vi "Is String Constant a State Constant.vi"(8 "error in (no error)":errorcluster, 11 "GObj Refnum":refnum<vi>) -> (0 "error out":errorcluster, 2 "Is States Constant":bool, 3 "Add States to Queue":refnum<vi>)   [LabVIEW 2020, in "JKI State Machine API.lvlib"]
uses:
  JKI State Machine API.lvlib
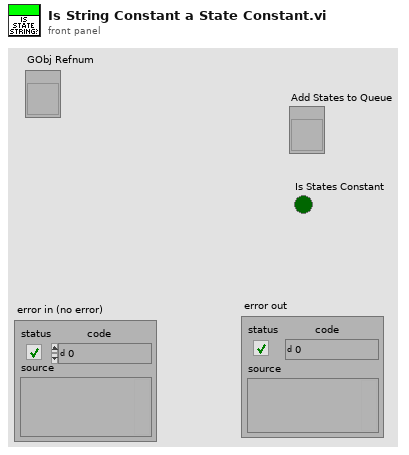
[diagram p1: front panel]
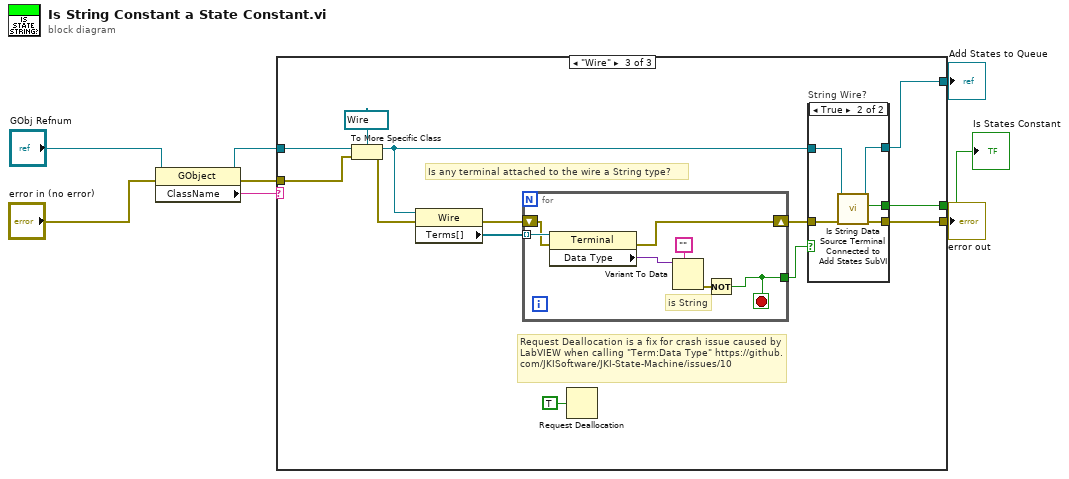
[diagram p0: block diagram]
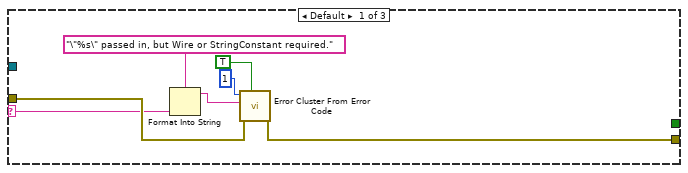
[diagram p2: hidden frame]
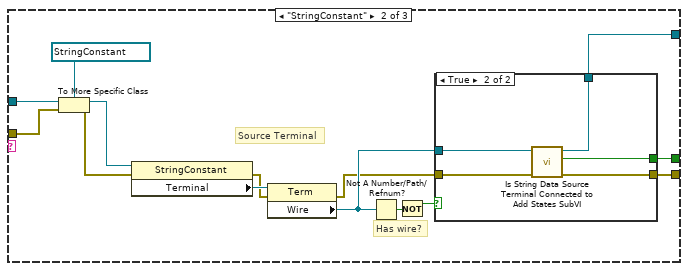
[diagram p3: hidden frame]
diagram:
  n1 = property class="GObject"(reference="GObj Refnum", error in="error in (no error)") -> (reference out=w4:refnum<vi>, error out=w2:errorcluster, "ClassName"=w1:string)
  n2 = case shown="\"Wire\"" w1 {
    selector: w1 -> [w13 _ _]
    tunnel: [w14 w29 w42] -> w8
    tunnel: [_ w28 w44] -> w7
    tunnel: [_ w27 w43] -> w6
    tunnel: w4 -> [_ w23 w46]
    tunnel: w2 -> [w15 w22 w45]
    frame Default {
      n3 = Format Into String(format string="\"%s\" passed in, but Wire or StringConstant required.", w13) -> (resulting string=w11:string)  [unwired: 2 in, 1 out]
      n4 = call <vilib>:"Error Cluster From Error Code.vi"("show call chain? (False)"=TRUE, "error in (no error)"=w15, "error message (\"\")"=w11, "error code (0)"=1) -> ("error out"=w14:errorcluster)  [unwired: 5 in]
    }
    frame "StringConstant" {
      # "Has wire?"
      # "Source Terminal"
      n5 = To More Specific Class(target class=refnum<vi> refnum ("StrCnst Refnum"), reference=w23, error in=w22) -> (specific class reference=w26:refnum<vi>, error out=w24:errorcluster)
      n6 = property class="StringConstant"(reference=w26, error in=w24) -> (error out=w17:errorcluster, "Terminal"=w21:refnum<vi>)  [unwired: 1 out]
      n7 = property class="Term"(reference=w21, error in=w17) -> (error out=w16:errorcluster, "Wire"=w18:refnum<vi>)  [unwired: 1 out]
      n8 = Not A Number/Path/Refnum?(number/path/refnum=w18) -> (NaN/Path/Refnum?=w20:bool)
      n9 = Not(x=w20) -> (.not. x?=w19:bool)
      n10 = case shown="True" w19 {
        tunnel: [w30 w35] -> w29
        tunnel: [_ w34] -> w28
        tunnel: w16 -> [w30 w33]
        tunnel: [_ w32] -> w27
        tunnel: w18 -> [_ w31]
        frame False {
        }
        frame True {
          n11 = call "Is String Data Source Terminal Connected to Add States SubVI.vi"("error in (no error)"=w33, "Wire"=w31) -> ("error out"=w35:errorcluster, "Connected to Add States?"=w34:bool, "Add States SubVI"=w32:refnum<vi>)  [unwired: 6 in, 1 out]
        }
      }
    }
    frame "Wire" {
      # "Request Deallocation is a fix for crash issue caused by LabVIEW when calling \"Term:Data Type\" https://github.com/JKISoftware/JKI-State-Machine/issues/10"
      # "Is any terminal attached to the wire a String type?"
      n12 = To More Specific Class(target class=refnum<vi> refnum ("Wire Refnum"), reference=w46, error in=w45) -> (specific class reference=w41:refnum<vi>, error out=w47:errorcluster)
      n13 = property class="Wire"(reference=w41, error in=w47) -> (error out=w40:errorcluster, "Terms[]"=w38:refnum<vi>[])  [unwired: 1 out]
      n14 = for {
        shift-right: [w59] -> w39
        shift-left: w40 -> [w60]
        tunnel: w38 -> [w61] mode=indexing
        tunnel: [w55] -> w37
        stop <- w55 stop-if-true
        # "is String"
        n15 = property class="Terminal"(reference=w61, error in=w60) -> (error out=w59:errorcluster, "Data Type"=w56:variant)  [unwired: 1 out]
        n16 = Variant To Data(type="" ("error in (no error)"), Variant=w56) -> (error out=w57:errorcluster)  [unwired: 1 in, 1 out]
        n17 = Not(x=w57) -> (.not. x?=w55:bool)
      }
      n18 = Request Deallocation(TRUE ("flag")) -> ()
      n19 = case "String Wire?" shown="True" w37 {
        tunnel: [_ w54] -> w44
        tunnel: [_ w53] -> w43
        tunnel: [w49 w52] -> w42
        tunnel: w41 -> [_ w51]
        tunnel: w39 -> [w49 w50]
        frame False {
        }
        frame True {
          n20 = call "Is String Data Source Terminal Connected to Add States SubVI.vi"("error in (no error)"=w50, "Wire"=w51) -> ("error out"=w52:errorcluster, "Connected to Add States?"=w54:bool, "Add States SubVI"=w53:refnum<vi>)  [unwired: 6 in, 1 out]
        }
      }
    }
  }
  "error out" <- w8
  "Is States Constant" <- w7
  "Add States to Queue" <- w6
